vi "eDyno TDMS Reducer.vi"(0 "Source TDMS Path":string="C:\\Users\\dihidalgÞsktop\\MCP\\MCP_SnV_TestÚta\\LogFile_2026-11-20-13-36-19.tdms", 5 "Output TDMS Path":string="C:\\Users\\dihidalgÞsktop\\MCP\\MCP_SnV_TestÚta\\Reduced_LogFile_2026-11-20-13-36-19.tdms", 7 "Snapshot Period (samples)":i32=768000, 9 "Snapshot Length (samples)":i32=51200) -> (4 "error out":errorcluster)   [LabVIEW 2026]
doc: "PURPOSE\nMakes a small copy of a large FlexLogger eDyno log so it can be reviewed or shared: every low-rate channel (CAN signals at 100 Hz and plug-in results at 10 Hz) is copied in full to group Log, and the two raw 51.2 kS/s channels (DSA_4464/ai0 accel in g, DAQ_6396/ai0 tach in V) are copied as short snapshots to group Raw (Accel_g, Tach_V).\n\nSNAPSHOTS\nSnapshot k starts at sample k x Snapshot Period and is Snapshot Length samples long; snapshots are appended back to back, so snapshot k occupies samples k x Length ... (k+1) x Length - 1 of the Raw channels. Defaults: 1 s every 15 s, 241 snapshots (whole 60 min log).\n\nOUTPUT\nOutput TDMS Path is created or replaced. Channels Copied = number of low-rate channels copied."
panel:
  out "Channels Copied":i32
  in  "Number of Snapshots":i32=241
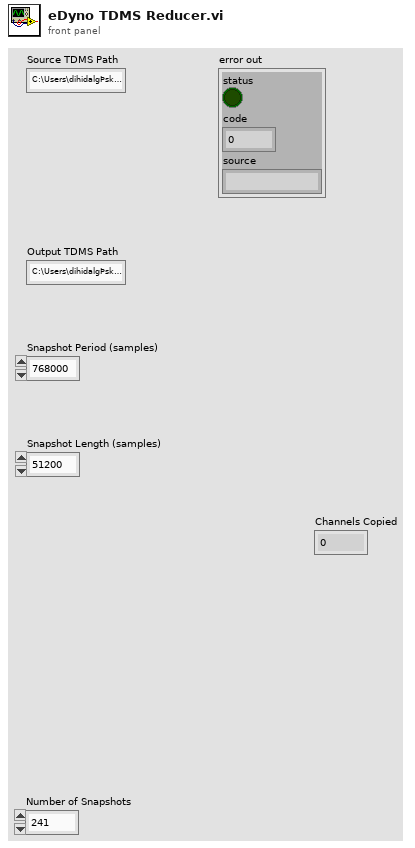
[diagram p1: front panel]
types:
  T1 = enum16{"open", "open or create", "create or replace", "create", "open (read-only)"}
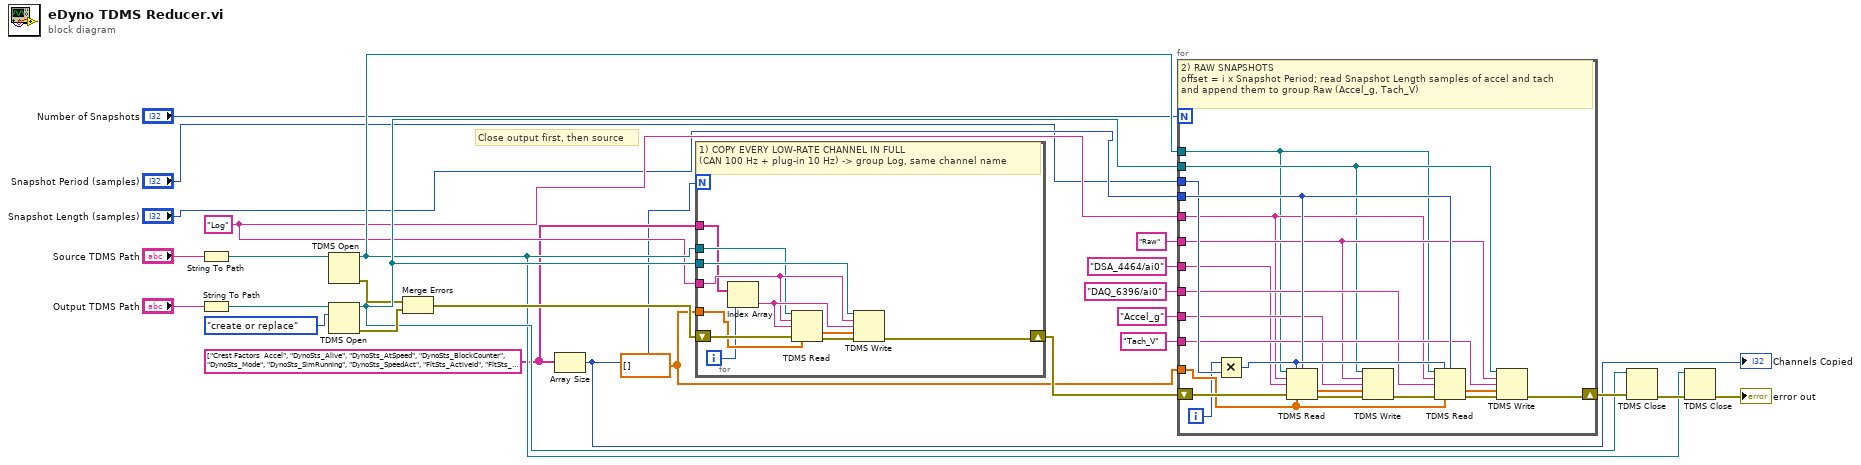
[diagram p0: block diagram]
diagram:
  w10 = "Log" ("group Log")
  w9 = dbl[] [] ("read as DBL")
  w8 = string[] ["Crest Factors  Accel", "DynoSts_Alive", "DynoSts_AtSpeed", "DynoSts_BlockCounter", "DynoSts_Mode", "DynoSts_SimRunning", "DynoSts_SpeedAct", "FltSts_ActiveId", "FltSts_Alive", "FltSts_BPFO_Amp", "FltSts_BPFO_On", "FltSts_Freq_1x", "FltSts_Freq_2x", "FltSts_Freq_BPFO", "FltSts_Freq_PWM", "FltSts_Freq_Ripple", "FltSts_Imbalance_Amp", "FltSts_Imbalance_On", "FltSts_Misalign_Amp", "FltSts_Misalign_On", "FltSts_PWM_Amp", "FltSts_PWM_On", "FltSts_Ripple_Amp", "FltSts_Ripple_On", "Kurtosis  Accel", "Max Level  Accel", "Max-Min Level   Accel", "MCU_ControllerTemp", "MCU_DCCurrent", "MCU_DCVoltage", "MCU_ElecPower", "MCU_MotorSpeed", "MCU_PhaseCurrentRms", "MCU_TorqueEst", "MCU_WindingTemp", "Min Level  Accel", "Peak Levels  Accel", "Powers in Band  Accel", "RMS Levels  Accel", "Skewness  Accel", "Velocity  Accel"] ("low-rate channels")
  # "Close output first, then source"
  n1 = String To Path(string="Source TDMS Path") -> (path=w17:path)
  n2 = String To Path(string="Output TDMS Path") -> (path=w18:path)
  n3 = TDMS Open(11:w17) -> (0:w20:errorcluster, 3:w19:refnum<k34>)  [unwired: 6 in]
  n4 = TDMS Open(10:T1."create or replace" ("create or replace"), 11:w18) -> (0:w22:errorcluster, 3:w21:refnum<k34>)  [unwired: 5 in]
  n5 = Merge Errors(w20, w22) -> (w23:errorcluster)
  n6 = Array Size(array=w8) -> (size(s)=w6:i32)
  "Channels Copied" <- w6
  n7 = for {
    N: w6 -> [_]
    tunnel: w8 -> [w28]
    tunnel: w9 -> [w31]
    tunnel: w10 -> [w32]
    tunnel: w19 -> [w29]
    tunnel: w21 -> [w30]
    shift-right: [w34] -> w24
    shift-left: w23 -> [w33]
    i -> [w27]
    # "1) COPY EVERY LOW-RATE CHANNEL IN FULL\n(CAN 100 Hz + plug-in 10 Hz) -> group Log, same channel name"
    n8 = Index Array(array=w28, index=w27) -> (element=w35:string)
    n9 = TDMS Read(0:w29, 5:w32, 7:w35, 11:w33, 12:w31) -> (10:w36:dbl[], 15:w37:errorcluster)  [unwired: 3 in, 4 out]
    n10 = TDMS Write(0:w30, 5:w32, 7:w35, 9:w36, 11:w37) -> (15:w34:errorcluster)  [unwired: 1 in, 3 out]
  }
  n11 = for {
    N: "Number of Snapshots" -> [_]
    tunnel: w9 -> [w41]
    tunnel: w10 -> [w42]
    tunnel: "Raw" ("group Raw") -> [w43]
    tunnel: "DSA_4464/ai0" ("raw accel") -> [w44]
    tunnel: "DAQ_6396/ai0" ("raw tach") -> [w45]
    tunnel: "Accel_g" ("out accel") -> [w46]
    tunnel: "Tach_V" ("out tach") -> [w47]
    tunnel: "Snapshot Period (samples)" -> [w48]
    tunnel: "Snapshot Length (samples)" -> [w49]
    tunnel: w19 -> [w39]
    tunnel: w21 -> [w40]
    shift-right: [w51] -> w25
    shift-left: w24 -> [w50]
    i -> [w38]
    # "2) RAW SNAPSHOTS\noffset = i x Snapshot Period; read Snapshot Length samples of accel and tach\nand append them to group Raw (Accel_g, Tach_V)"
    n12 = Multiply(x=w38, y=w48) -> (x*y=w52:i32)
    n13 = TDMS Read(0:w39, 1:w52, 2:w49, 5:w42, 7:w44, 11:w50, 12:w41) -> (10:w53:dbl[], 15:w54:errorcluster)  [unwired: 1 in, 4 out]
    n14 = TDMS Write(0:w40, 5:w43, 7:w46, 9:w53, 11:w54) -> (15:w55:errorcluster)  [unwired: 1 in, 3 out]
    n15 = TDMS Read(0:w39, 1:w52, 2:w49, 5:w42, 7:w45, 11:w55, 12:w41) -> (10:w56:dbl[], 15:w57:errorcluster)  [unwired: 1 in, 4 out]
    n16 = TDMS Write(0:w40, 5:w43, 7:w47, 9:w56, 11:w57) -> (15:w51:errorcluster)  [unwired: 1 in, 3 out]
  }
  n17 = TDMS Close(8:w25, 11:w21) -> (0:w26:errorcluster)  [unwired: 1 out]
  n18 = TDMS Close(8:w26, 11:w19) -> (0:→"error out":errorcluster)  [unwired: 1 out]
